vi "CSE - Diagnose Statement.vi"(6 "sort (F)":bool, 8 "error in":errorcluster, 9 "Items":i32(ring) items=["Variables", "Functions", "FuncVI functions", "FastFunc functions"], 10 "Stm Index":i32, 11 "CSE RefNum":T1) -> (0 "error out":errorcluster, 1 "Array of Items":string[](array[string]), 2 "dup Stm Index":i32, 3 "dup CSE RefNum":T1, 4 "Original List of Items":string, 5 "expression":bool)   [LabVIEW 2021]
doc: "This VI returns the names of variables and functions referenced in the specified statement of a parsed script. Refer to the VI help for more details.\n\n::: CalcExpress Toolkit :::\nCopyright (c) 2000-2026 Konstantin Shifershteyn. All rights reserved."
uses:
  CSE Instance RefNum.ctl
  cersrc/celveng32.dll
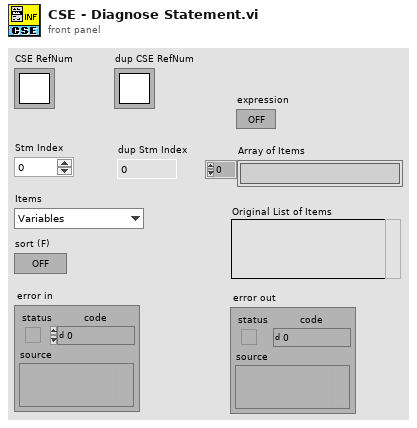
[diagram p1: front panel]
types:
  T1 = typedef "CSE Instance RefNum.ctl" = refnum<k1>
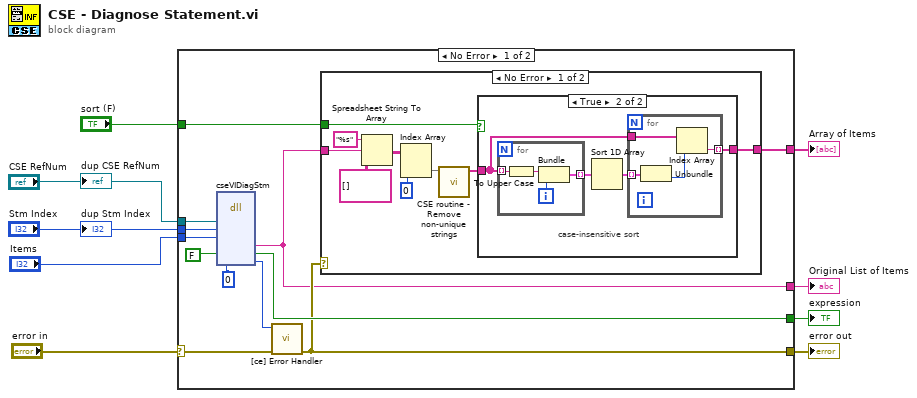
[diagram p0: block diagram]
diagram:
  n1 = case shown="No Error" "error in" {
    selector: "error in" -> [w18 w44]
    tunnel: "Stm Index" -> [w21 _]
    tunnel: "CSE RefNum" -> [w20 _]
    tunnel: [w12 w44] -> w7
    tunnel: "Items" -> [w19 _]
    tunnel: [w13 _] -> w4
    tunnel: [w11 _] -> w3
    tunnel: [w14 _] -> w2
    tunnel: "sort (F)" -> [w10 _]
    frame No Error {
      n2 = dll-call lib="C:/LV Projects/CalcExpress 40 LV2021/vi.lib/addons/CalcExpress/cersrc/celveng*.dll" fn="cseVIDiagStm"("iCESP"=w20, "StmIndex"=w21, "ItemID"=w19, "express"=FALSE, "errStat"=0) -> ("outString"=w11:string, "express"=w14:bool, "errStat"=w15:i32)  [unwired: 8 in, 2 out]
      n3 = call "[ce] Error Handler.vi"("error in"=w18, "error code"=w15) -> ("error out"=w12:errorcluster)  [unwired: 8 in, 1 out]
      n4 = case shown="No Error" w12 {
        tunnel: [w29 _] -> w13
        tunnel: w10 -> [w28 _]
        tunnel: w11 -> [w22 _]
        frame No Error {
          n5 = Spreadsheet String To Array(format string="%s", spreadsheet string=w22, array type (2D Dbl)=string[][] []) -> (array=w25:string[][])  [unwired: 1 in]
          n6 = Index Array(array=w25, index (col)=0 ("disabled index (col)")) -> (element=w23:string[])  [unwired: 1 in]
          n7 = call "CSE routine - Remove non-unique strings.vi"("Array in"=w23) -> ("Array out"=w30:string[])  [unwired: 7 in, 1 out]
          n8 = case shown="True" w28 {
            tunnel: w30 -> [w31 w33]
            tunnel: [w31 w32] -> w29
            frame False {
            }
            frame True {
              # "case-insensitive sort"
              n9 = for {
                tunnel: w33 -> [w42] mode=indexing
                tunnel: [w40] -> w35 mode=indexing
                i -> [w43]
                n10 = To Upper Case(1:w42) -> (0:w41:string)
                n11 = Bundle(w41, w43) -> (w40:cluster{string, i32})  [unwired: 1 in]
              }
              n12 = Sort 1D Array(array=w35) -> (sorted array=w34:cluster{string, i32}[])
              n13 = for {
                tunnel: w34 -> [w39] mode=indexing
                tunnel: w33 -> [w38]
                tunnel: [w36] -> w32 mode=indexing
                n14 = Unbundle(w39) -> (w37:i32)  [unwired: 1 out]
                n15 = Index Array(array=w38, index=w37) -> (element=w36:string)
              }
            }
          }
        }
        frame Error {
        }
      }
    }
    frame Error {
    }
  }
  "error out" <- w7
  "Array of Items" <- w4
  "Original List of Items" <- w3
  "expression" <- w2
  "dup Stm Index" <- "Stm Index"
  "dup CSE RefNum" <- "CSE RefNum"
